vi "_lcod_CFX.vi"(4 "RequestTargetAddress":string="rabbit@SMT-001", 6 "RequestNetworkUri":string="amqp://localhost:5672/#/connections.com", 7 "cmd":T2, 8 "Error In":errorcluster caption="错误输入", 9 "in_str":string, 10 "CFXHandle":string="SDC.SMT.001", 11 "CfxData":T1) -> (0 "Error Out":errorcluster caption="错误输出", 2 "MessageName":string, 3 "new reference":refnum<k24>)   [LabVIEW 2025]
uses:
  ctl/CfxTopic-cmd.ctl
  CFX_dll/CFX.dll
  ctl/CFX_data.ctl
  <vilib>/Utility/error.llb/Trim Whitespace One-Sided.vi
panel:
  out "FaultOccurrenceId":string
  out "ToJson":string
  out "Message":string
  in  "Uri":string="amqp://localhost:5672/#/connections.com:5672"
  # "EndpointInformation/RequestResult/SupportedTopics"
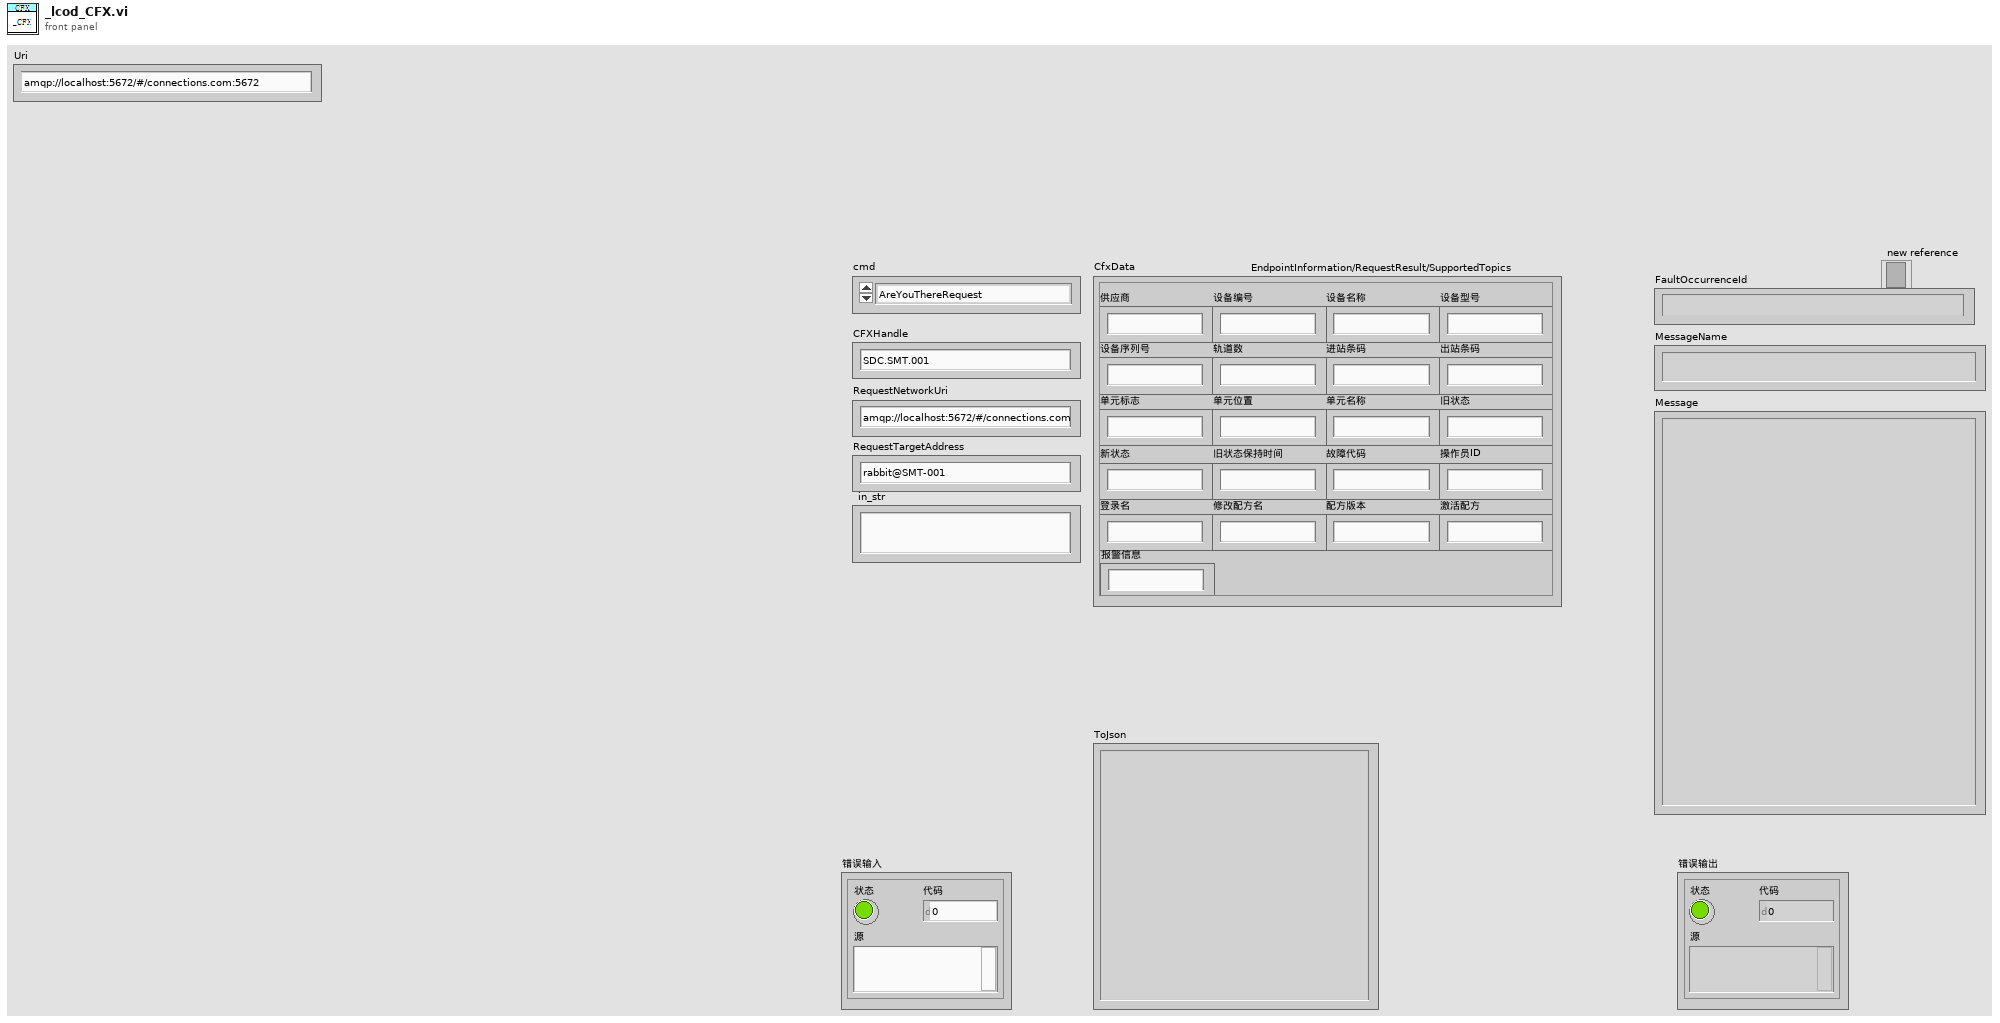
[diagram p1: front panel]
types:
  T1 = typedef "CFX_data.ctl" = cluster{"Vendor":string, "UniqueIdentifier":string, "FriendlyName":string, "ModelNumber":string, "SerialNumber":string, "NumberofLanes":string, "CodeIn":string, "CodeOut":string, "Unitldentifer":string, "PositionNumber":string, "PositionName":string, "OldState":string, "NewState":string, "OldStateDuration":string, "Faultcode":string, "Operatorldentifer":string, "LoginName":string, "RecipeName":string, "Revision":string, "Activate formula":string, "Description":string}
  T2 = typedef "CfxTopic-cmd.ctl" = enum16{"AreYouThereRequest", "AreYouThereResponse", "EndpointConnected", "EndpointShuttingDown", "GetEndpointInformationRequest", "GetEndpointInformationResponse", "Heartbeat", "NotSupportedResponse", "WhoIsThereRequest", "WhoIsThereResponse", "UnitArrived", "UnitsDeparted", "StationStateChanged", "FaultOccurred", "FaultCleared", "OperatorActivated", "OperatorDeactivated", "RecipeModified", "RecipeActived", "ActivateRecipeRequest", "ActivateRecipeResponse"}
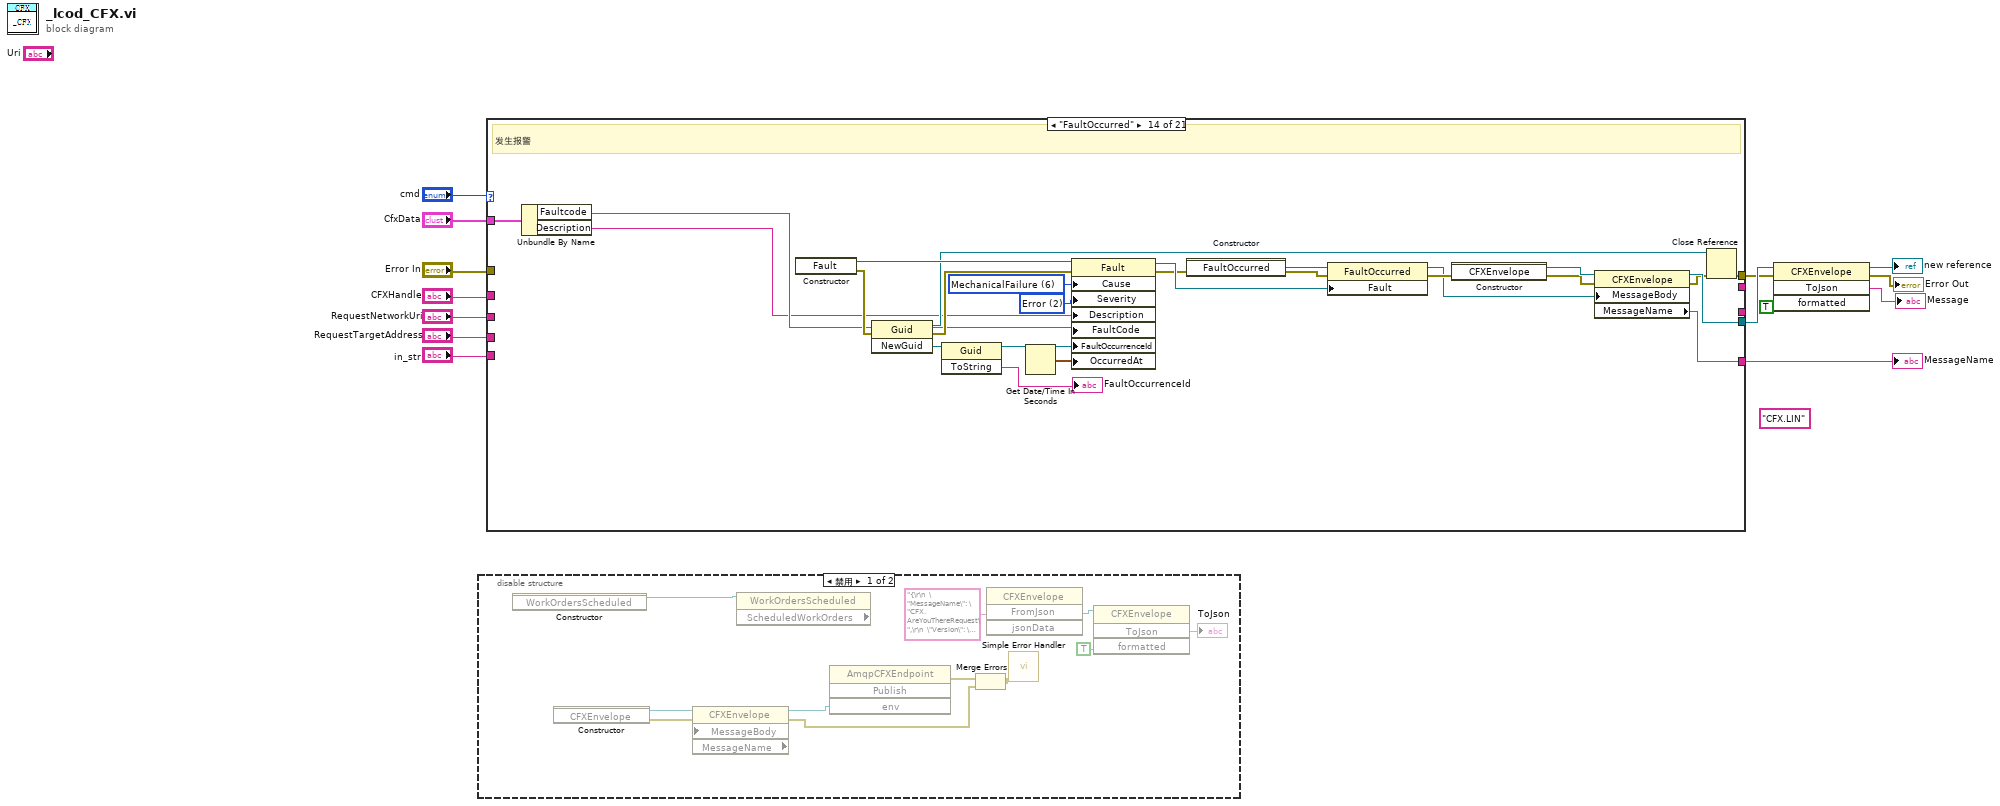
[diagram p0: block diagram]
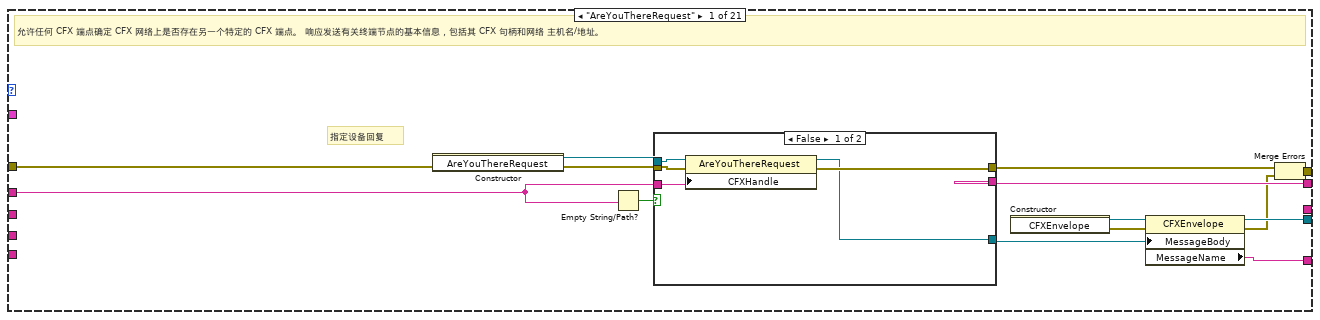
[diagram p3: hidden frame]
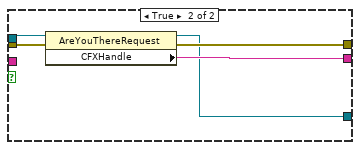
[diagram p4: hidden frame]
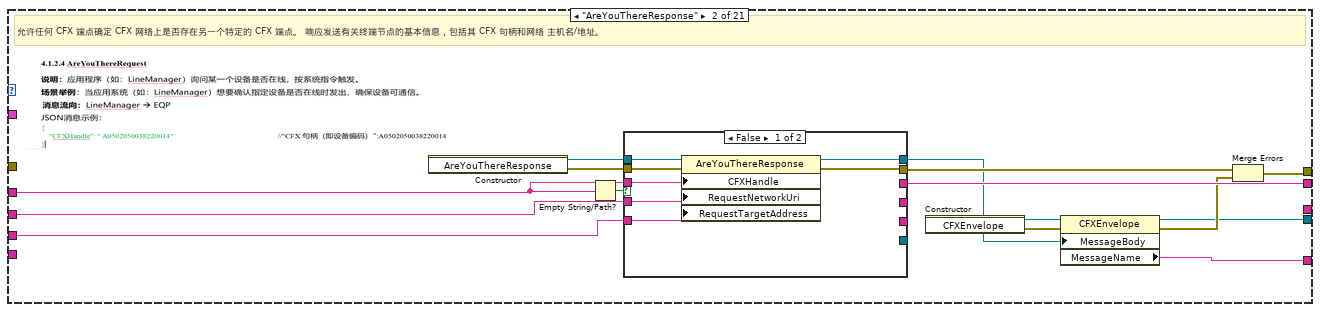
[diagram p5: hidden frame]
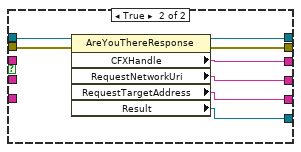
[diagram p6: hidden frame]
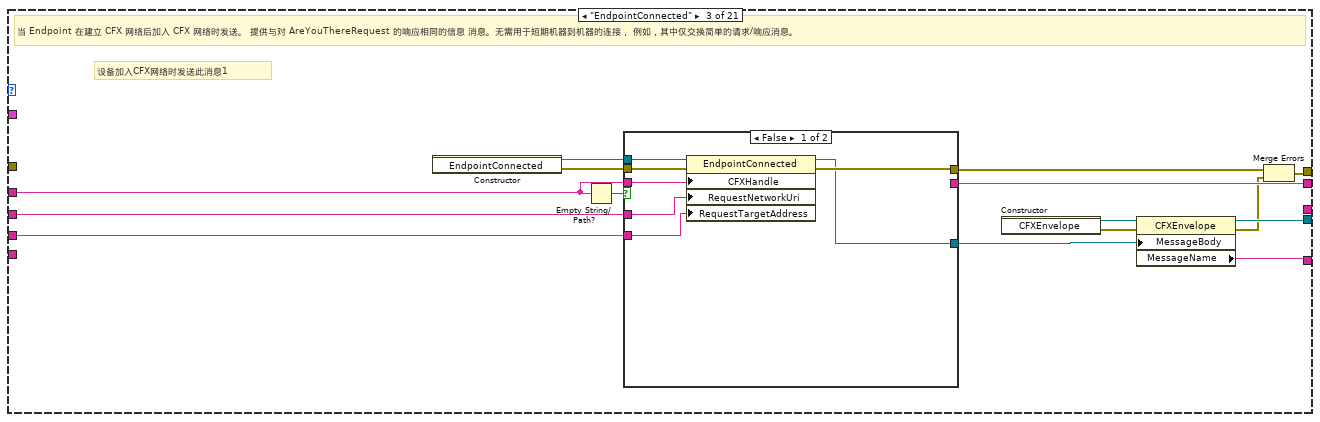
[diagram p7: hidden frame]
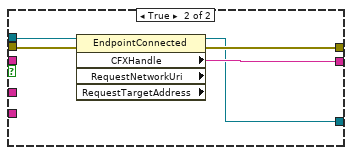
[diagram p8: hidden frame]
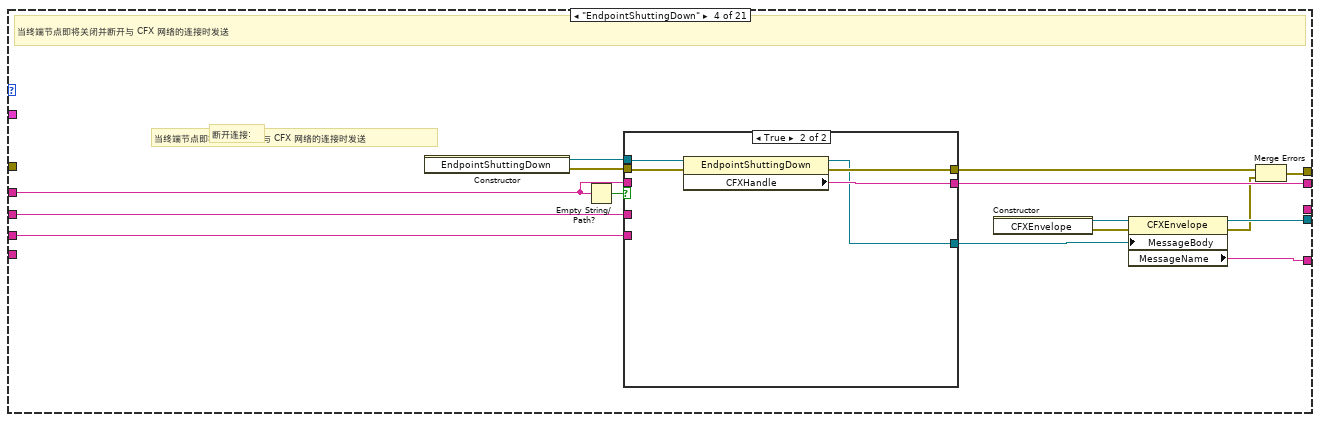
[diagram p9: hidden frame]
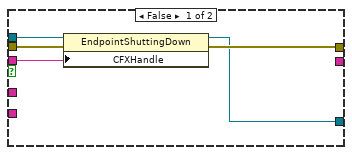
[diagram p10: hidden frame]
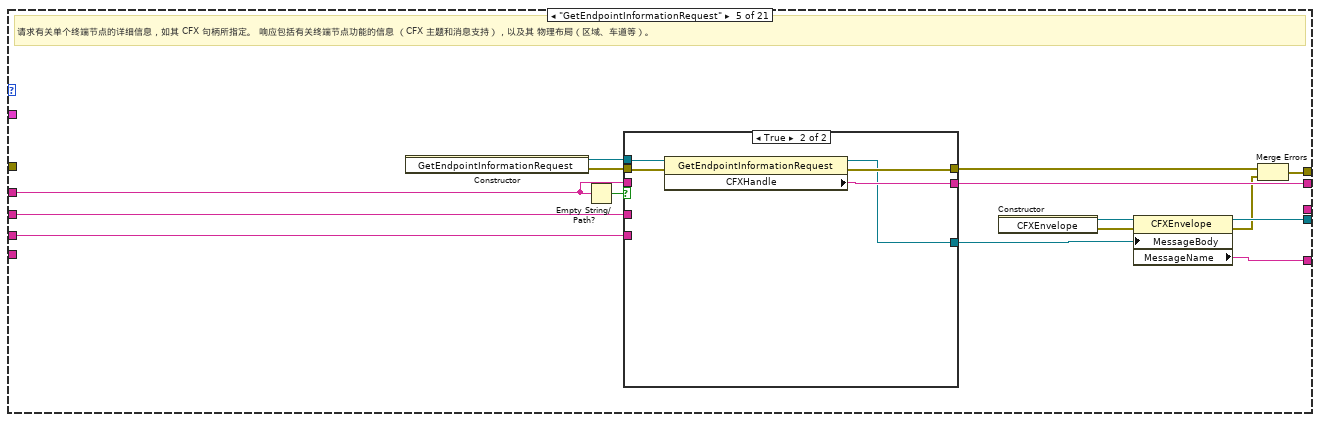
[diagram p11: hidden frame]
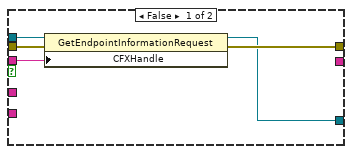
[diagram p12: hidden frame]
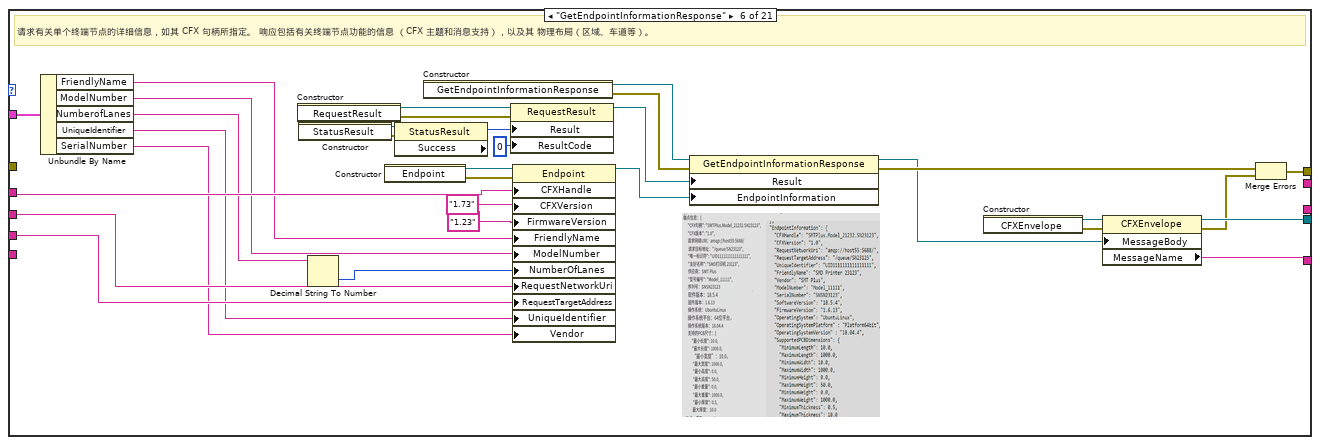
[diagram p13: hidden frame]
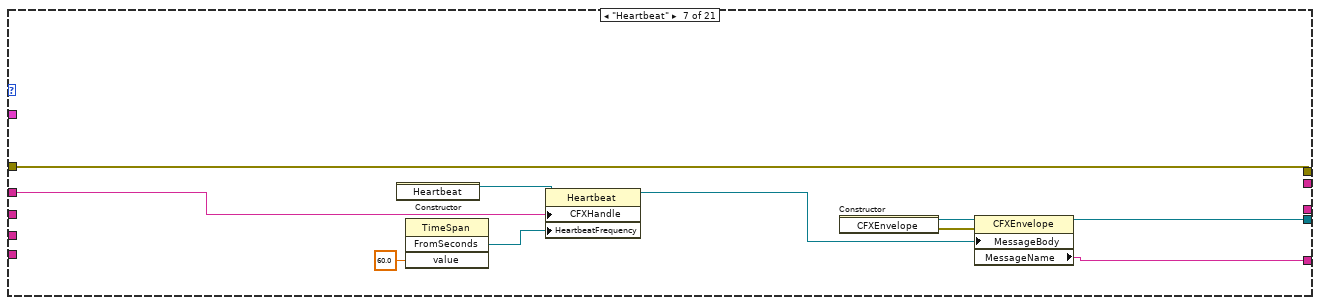
[diagram p14: hidden frame]
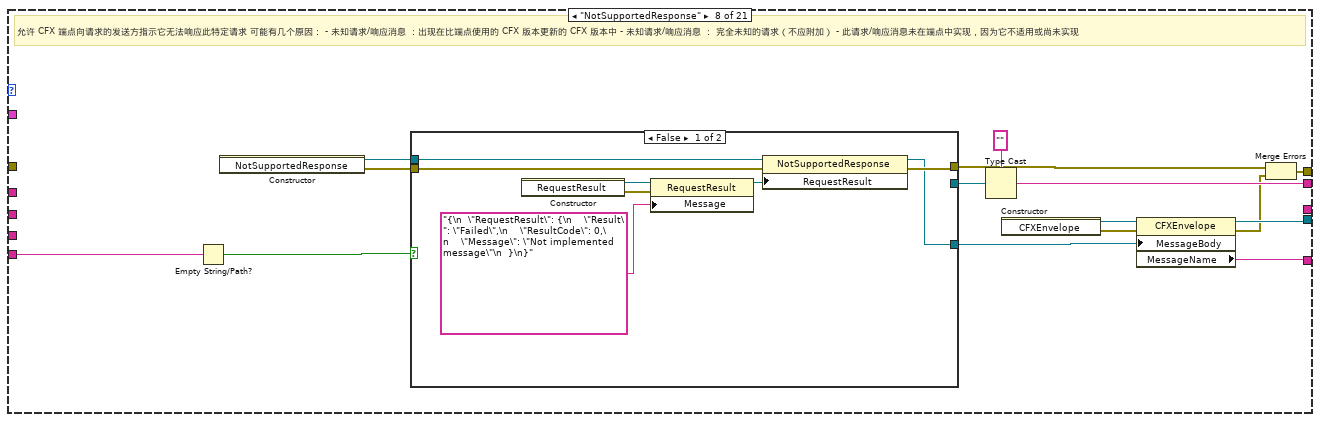
[diagram p15: hidden frame]
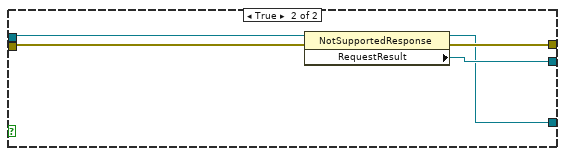
[diagram p16: hidden frame]
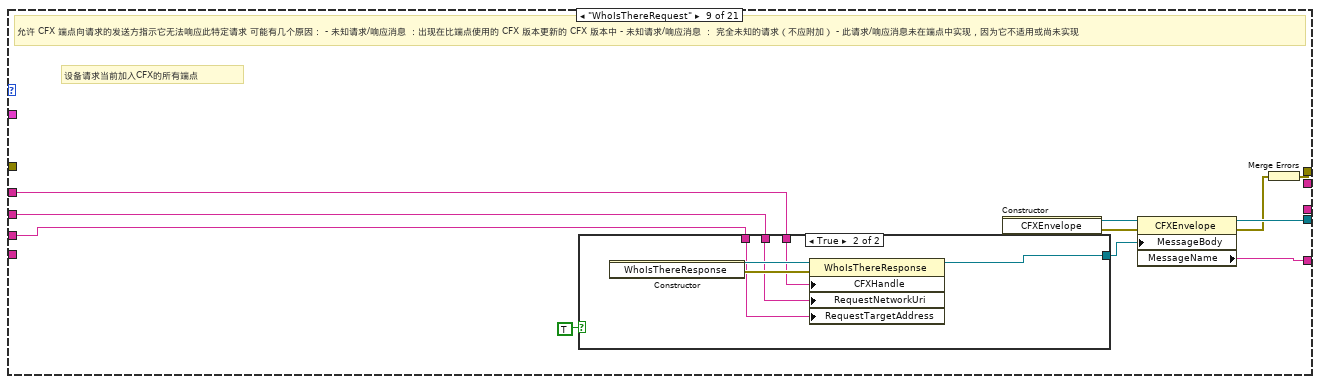
[diagram p17: hidden frame]
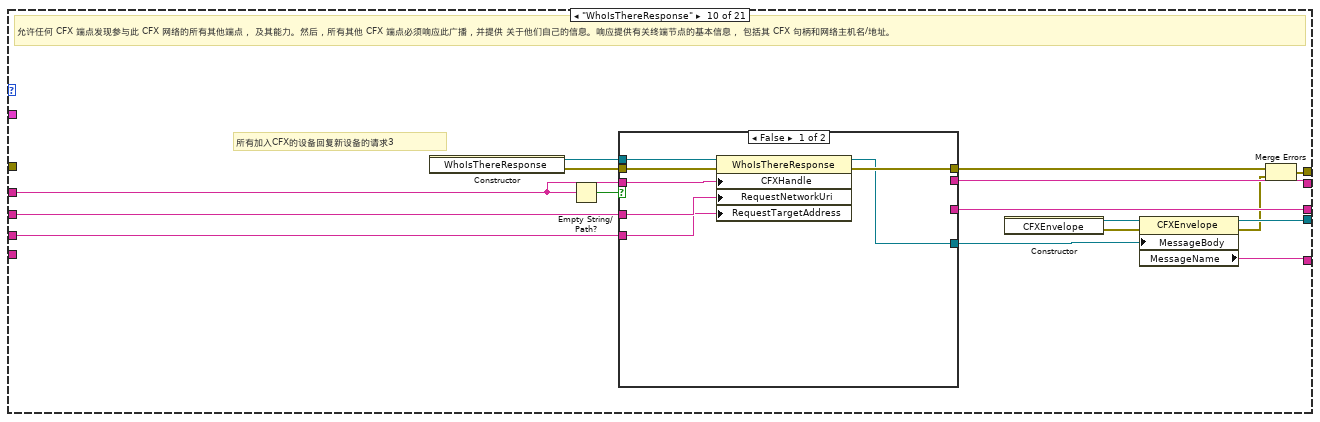
[diagram p19: hidden frame]
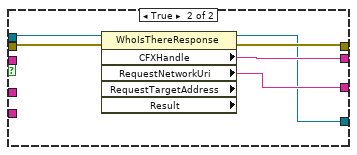
[diagram p20: hidden frame]
diagram:
  (unwired) "CFX.LIN" ("messageType")
  n1 = disable-structure shown="禁用" {
    frame Disabled {
      n2 = constructor class="WorkOrdersScheduled"() -> (reference out=w25:refnum<k24>)  [unwired: 3 in, 2 out]
      n3 = constructor class="CFXEnvelope"() -> (reference out=w22:refnum<k24>, error out=w21:errorcluster)  [unwired: 3 in, 1 out]
      n4 = property class="CFXEnvelope" props=["MessageBody", "MessageName"](reference=w22, error in=w21) -> (reference out=w20:refnum<k24>, error out=w24:errorcluster)  [unwired: 1 in, 1 out]
      n5 = property class="WorkOrdersScheduled" props=["ScheduledWorkOrders"](reference=w25) -> ()  [unwired: 1 in, 3 out]
      n6 = invoke class="AmqpCFXEndpoint" method="Publish"("env"=w20) -> (error out=w19:errorcluster)  [unwired: 3 in, 3 out]
      n7 = Merge Errors(w19, w24) -> (w23:errorcluster)
      n8 = invoke class="CFXEnvelope" method="FromJson"("jsonData"="{\r\n  \"MessageName\": \"CFX.AreYouThereRequest\",\r\n  \"Version\": \"1.75\",\r\n  \"TimeStamp\": \"2025-10-18T15:23:20.890711+08:00\",\r\n  \"UniqueID\": \"92a07db6-b3a6-406f-a014-7739e04793a1\",\r\n  \"Source\": null,\r\n  \"Target\": null,\r\n  \"RequestID\": null,\r\n  \"MessageBody\": {\n\n  \"$type\": \"CFX.AreYouThereRequest, CFX\",\r\n    \"CFXHandle\": \"SDC.SMT.001\"\n\r\n  }\r\n}" ("ToJson")) -> ("FromJson"=w18:refnum<k24>)  [unwired: 3 in, 3 out]
      n9 = call <vilib>:"Simple Error Handler.vi"("error in (no error)"=w23) -> ()  [unwired: 4 in, 5 out]
      n10 = invoke class="CFXEnvelope" method="ToJson"(reference=w18, "formatted"=TRUE) -> ("ToJson"=→"ToJson":string)  [unwired: 2 in, 3 out]
    }
    frame Enabled {
    }
  }
  n11 = case shown="\"FaultOccurred\"" "cmd" {
    tunnel: [w36 w61 w92 w119 w144 _ _ w208 _ w252 _ _ _ _ _ _ _ _ _ _ _] -> _
    tunnel: "CFXHandle" -> [w35 w60 w90 w117 w142 w165 w196 _ w228 w255 _ _ _ _ _ _ _ _ _ _ _]
    tunnel: [w27 w53 w82 w109 w134 w181 w198 w201 w234 w246 w292 w312 w346 w373 w397 w425 w439 w458 w471 w486 w494] -> w4
    tunnel: "Error In" -> [w33 _ _ _ _ _ w198 _ _ _ _ _ _ _ _ _ _ _ w475 _ _]
    tunnel: "RequestTargetAddress" -> [_ w59 w88 w115 w140 w168 _ _ w227 w253 _ _ _ _ _ _ _ _ _ _ _]
    tunnel: "RequestNetworkUri" -> [_ w58 w89 w116 w141 w169 _ _ w229 w254 _ _ _ _ _ _ _ _ _ _ _]
    tunnel: "in_str" -> [_ _ _ _ _ _ _ w209 _ _ _ _ _ _ _ _ _ _ _ _ _]
    tunnel: [_ _ _ _ _ _ _ _ _ w251 _ _ _ _ _ _ _ _ _ _ _] -> _
    tunnel: [w29 w51 w83 w111 w136 w183 w193 w203 w235 w248 w294 w311 w347 w381 w409 w421 w438 w457 w473 w485 w498] -> w6
    tunnel: [w28 w50 w80 w107 w132 w179 w189 w199 w232 w244 w290 w310 w343 w379 w406 w423 w437 w456 w472 w484 w497] -> w8
    tunnel: "CfxData" -> [_ _ _ _ _ w164 _ _ _ _ w280 w308 w342 w378 w405 w420 w436 w453 w470 w483 _]
    frame "AreYouThereRequest" {
      # "指定设备回复"
      # "允许任何 CFX 端点确定 CFX 网络上是否存在另一个特定的 CFX 端点。 响应发送有关终端节点的基本信息，包括其 CFX 句柄和网络 主机名/地址。"
      n12 = constructor class="AreYouThereRequest"(error in=w33) -> (reference out=w38:refnum<k24>, error out=w39:errorcluster)  [unwired: 2 in, 1 out]
      n13 = Empty String/Path?(string/path=w35) -> (empty?=w37:bool)
      n14 = case shown="False" w37 {
        tunnel: w39 -> [w44 w47]
        tunnel: w35 -> [w43 _]
        tunnel: w38 -> [w42 w49]
        tunnel: [_ w48] -> w36
        tunnel: [w41 w46] -> w34
        tunnel: [w40 w45] -> w30
        frame False {
          n15 = property class="AreYouThereRequest"(reference=w42, error in=w44, "CFXHandle"=w43) -> (reference out=w40:refnum<k24>, error out=w41:errorcluster)
        }
        frame True {
          n16 = property class="AreYouThereRequest"(reference=w49, error in=w47) -> (reference out=w45:refnum<k24>, error out=w46:errorcluster, "CFXHandle"=w48:string)
        }
      }
      n17 = constructor class="CFXEnvelope"() -> (reference out=w32:refnum<k24>, error out=w31:errorcluster)  [unwired: 3 in, 1 out]
      n18 = property class="CFXEnvelope"(reference=w32, error in=w31, "MessageBody"=w30) -> (reference out=w29:refnum<k24>, error out=w26:errorcluster, "MessageName"=w28:string)
      n19 = Merge Errors(w34, w26) -> (w27:errorcluster)
    }
    frame "AreYouThereResponse" {
      # "允许任何 CFX 端点确定 CFX 网络上是否存在另一个特定的 CFX 端点。 响应发送有关终端节点的基本信息，包括其 CFX 句柄和网络 主机名/地址。"
      n20 = constructor class="AreYouThereResponse"() -> (reference out=w63:refnum<k24>, error out=w64:errorcluster)  [unwired: 3 in, 1 out]
      n21 = Empty String/Path?(string/path=w60) -> (empty?=w62:bool)
      n22 = case shown="False" w62 {
        tunnel: w64 -> [w71 w77]
        tunnel: w60 -> [w70 _]
        tunnel: w63 -> [w69 w79]
        tunnel: [_ w78] -> w61
        tunnel: w58 -> [w68 _]
        tunnel: w59 -> [w67 _]
        tunnel: [_ w76] -> _
        tunnel: [_ w75] -> _
        tunnel: [_ w74] -> _
        tunnel: [w66 w73] -> w57
        tunnel: [w65 w72] -> w54
        frame False {
          n23 = property class="AreYouThereResponse"(reference=w69, error in=w71, "CFXHandle"=w70, "RequestNetworkUri"=w68, "RequestTargetAddress"=w67) -> (reference out=w65:refnum<k24>, error out=w66:errorcluster)
        }
        frame True {
          n24 = property class="AreYouThereResponse"(reference=w79, error in=w77) -> (reference out=w72:refnum<k24>, error out=w73:errorcluster, "CFXHandle"=w78:string, "RequestNetworkUri"=w76:string, "RequestTargetAddress"=w75:string, "Result"=w74:refnum<k24>)
        }
      }
      n25 = constructor class="CFXEnvelope"() -> (reference out=w56:refnum<k24>, error out=w55:errorcluster)  [unwired: 3 in, 1 out]
      n26 = property class="CFXEnvelope"(reference=w56, error in=w55, "MessageBody"=w54) -> (reference out=w51:refnum<k24>, error out=w52:errorcluster, "MessageName"=w50:string)
      n27 = Merge Errors(w57, w52) -> (w53:errorcluster)
    }
    frame "EndpointConnected" {
      # "设备加入CFX网络时发送此消息1"
      # "当 Endpoint 在建立 CFX 网络后加入 CFX 网络时发送。 提供与对 AreYouThereRequest 的响应相同的信息 消息。无需用于短期机器到机器的连接， 例如，其中仅交换简单的请求/响应消息。"
      n28 = constructor class="EndpointConnected"() -> (reference out=w93:refnum<k24>, error out=w94:errorcluster)  [unwired: 3 in, 1 out]
      n29 = Empty String/Path?(string/path=w90) -> (empty?=w91:bool)
      n30 = case shown="False" w91 {
        tunnel: w94 -> [w101 w105]
        tunnel: w93 -> [w100 w106]
        tunnel: [_ w104] -> w92
        tunnel: w90 -> [w99 _]
        tunnel: w89 -> [w96 _]
        tunnel: w88 -> [w95 _]
        tunnel: [w98 w103] -> w87
        tunnel: [w97 w102] -> w84
        frame False {
          n31 = property class="EndpointConnected"(reference=w100, error in=w101, "CFXHandle"=w99, "RequestNetworkUri"=w96, "RequestTargetAddress"=w95) -> (reference out=w97:refnum<k24>, error out=w98:errorcluster)
        }
        frame True {
          n32 = property class="EndpointConnected" props=["CFXHandle", "RequestNetworkUri", "RequestTargetAddress"](reference=w106, error in=w105) -> (reference out=w102:refnum<k24>, error out=w103:errorcluster, "CFXHandle"=w104:string)  [unwired: 2 out]
        }
      }
      n33 = constructor class="CFXEnvelope"() -> (reference out=w86:refnum<k24>, error out=w85:errorcluster)  [unwired: 3 in, 1 out]
      n34 = property class="CFXEnvelope"(reference=w86, error in=w85, "MessageBody"=w84) -> (reference out=w83:refnum<k24>, error out=w81:errorcluster, "MessageName"=w80:string)
      n35 = Merge Errors(w87, w81) -> (w82:errorcluster)
    }
    frame "EndpointShuttingDown" {
      # "当终端节点即将关闭并断开与 CFX 网络的连接时发送"
      # "断开连接:"
      # "当终端节点即将关闭并断开与 CFX 网络的连接时发送"
      n36 = constructor class="EndpointShuttingDown"() -> (reference out=w120:refnum<k24>, error out=w121:errorcluster)  [unwired: 3 in, 1 out]
      n37 = Empty String/Path?(string/path=w117) -> (empty?=w118:bool)
      n38 = case shown="True" w118 {
        tunnel: w121 -> [w126 w130]
        tunnel: w120 -> [w125 w131]
        tunnel: [_ w129] -> w119
        tunnel: w117 -> [w124 _]
        tunnel: w116 -> [_ _]
        tunnel: w115 -> [_ _]
        tunnel: [w123 w128] -> w114
        tunnel: [w122 w127] -> w110
        frame False {
          n39 = property class="EndpointShuttingDown"(reference=w125, error in=w126, "CFXHandle"=w124) -> (reference out=w122:refnum<k24>, error out=w123:errorcluster)
        }
        frame True {
          n40 = property class="EndpointShuttingDown"(reference=w131, error in=w130) -> (reference out=w127:refnum<k24>, error out=w128:errorcluster, "CFXHandle"=w129:string)
        }
      }
      n41 = constructor class="CFXEnvelope"() -> (reference out=w113:refnum<k24>, error out=w112:errorcluster)  [unwired: 3 in, 1 out]
      n42 = property class="CFXEnvelope"(reference=w113, error in=w112, "MessageBody"=w110) -> (reference out=w111:refnum<k24>, error out=w108:errorcluster, "MessageName"=w107:string)
      n43 = Merge Errors(w114, w108) -> (w109:errorcluster)
    }
    frame "GetEndpointInformationRequest" {
      # "请求有关单个终端节点的详细信息，如其 CFX 句柄所指定。 响应包括有关终端节点功能的信息 （CFX 主题和消息支持），以及其 物理布局（区域、车道等）。"
      n44 = constructor class="GetEndpointInformationRequest"() -> (reference out=w145:refnum<k24>, error out=w146:errorcluster)  [unwired: 3 in, 1 out]
      n45 = Empty String/Path?(string/path=w142) -> (empty?=w143:bool)
      n46 = case shown="True" w143 {
        tunnel: w146 -> [w151 w155]
        tunnel: w145 -> [w150 w156]
        tunnel: [_ w154] -> w144
        tunnel: w142 -> [w149 _]
        tunnel: w141 -> [_ _]
        tunnel: w140 -> [_ _]
        tunnel: [w148 w153] -> w139
        tunnel: [w147 w152] -> w135
        frame False {
          n47 = property class="GetEndpointInformationRequest"(reference=w150, error in=w151, "CFXHandle"=w149) -> (reference out=w147:refnum<k24>, error out=w148:errorcluster)
        }
        frame True {
          n48 = property class="GetEndpointInformationRequest"(reference=w156, error in=w155) -> (reference out=w152:refnum<k24>, error out=w153:errorcluster, "CFXHandle"=w154:string)
        }
      }
      n49 = constructor class="CFXEnvelope"() -> (reference out=w138:refnum<k24>, error out=w137:errorcluster)  [unwired: 3 in, 1 out]
      n50 = property class="CFXEnvelope"(reference=w138, error in=w137, "MessageBody"=w135) -> (reference out=w136:refnum<k24>, error out=w133:errorcluster, "MessageName"=w132:string)
      n51 = Merge Errors(w139, w133) -> (w134:errorcluster)
    }
    frame "GetEndpointInformationResponse" {
      # "请求有关单个终端节点的详细信息，如其 CFX 句柄所指定。 响应包括有关终端节点功能的信息 （CFX 主题和消息支持），以及其 物理布局（区域、车道等）。"
      n52 = Unbundle By Name(w164) -> ("FriendlyName"=w162:string, "ModelNumber"=w161:string, "NumberofLanes"=w160:string, "UniqueIdentifier"=w159:string, "SerialNumber"=w158:string)
      n53 = constructor class="RequestResult"() -> (reference out=w178:refnum<k24>, error out=w177:errorcluster)  [unwired: 3 in, 1 out]
      n54 = constructor class="StatusResult"() -> (reference out=w176:refnum<k24>, error out=w175:errorcluster)  [unwired: 3 in, 1 out]
      n55 = Decimal String To Number(string=w160) -> (number=w157:i32)  [unwired: 2 in, 1 out]
      n56 = constructor class="Endpoint"() -> (reference out=w163:refnum<k24>, error out=w172:errorcluster)  [unwired: 3 in, 1 out]
      n57 = property class="StatusResult"(reference=w176, error in=w175) -> ("Success"=w174:i32)  [unwired: 2 out]
      n58 = constructor class="GetEndpointInformationResponse"() -> (reference out=w187:refnum<k24>, error out=w188:errorcluster)  [unwired: 3 in, 1 out]
      n59 = property on="属性节点" class="RequestResult"(reference=w178, error in=w177, "Result"=w174, "ResultCode"=0) -> (reference out=w167:refnum<k24>)  [unwired: 1 out]
      n60 = property class="Endpoint"(reference=w163, error in=w172, "CFXHandle"=w165, "CFXVersion"="1.73", "FirmwareVersion"="1.23", "FriendlyName"=w162, "ModelNumber"=w161, "NumberOfLanes"=w157, "RequestNetworkUri"=w169, "RequestTargetAddress"=w168, "UniqueIdentifier"=w159, "Vendor"=w158) -> (reference out=w166:refnum<k24>)  [unwired: 1 out]
      n61 = property class="GetEndpointInformationResponse"(reference=w187, error in=w188, "Result"=w167, "EndpointInformation"=w166) -> (reference out=w182:refnum<k24>, error out=w186:errorcluster)
      n62 = constructor class="CFXEnvelope"() -> (reference out=w185:refnum<k24>, error out=w184:errorcluster)  [unwired: 3 in, 1 out]
      n63 = property class="CFXEnvelope"(reference=w185, error in=w184, "MessageBody"=w182) -> (reference out=w183:refnum<k24>, error out=w180:errorcluster, "MessageName"=w179:string)
      n64 = Merge Errors(w186, w180) -> (w181:errorcluster)
    }
    frame "Heartbeat" {
      n65 = constructor class="Heartbeat"() -> (reference out=w197:refnum<k24>)  [unwired: 3 in, 2 out]
      n66 = invoke on="调用节点" class="TimeSpan" method="FromSeconds"("value"=60.0) -> ("FromSeconds"=w191:refnum<k24>)  [unwired: 3 in, 3 out]
      n67 = property class="Heartbeat"(reference=w197, "CFXHandle"=w196, "HeartbeatFrequency"=w191) -> (reference out=w192:refnum<k24>)  [unwired: 1 in, 1 out]
      n68 = constructor class="CFXEnvelope"() -> (reference out=w195:refnum<k24>, error out=w194:errorcluster)  [unwired: 3 in, 1 out]
      n69 = property class="CFXEnvelope"(reference=w195, error in=w194, "MessageBody"=w192) -> (reference out=w193:refnum<k24>, "MessageName"=w189:string)  [unwired: 1 out]
    }
    frame "NotSupportedResponse" {
      # "允许 CFX 端点向请求的发送方指示它无法响应此特定请求 可能有几个原因： - 未知请求/响应消息 ：出现在比端点使用的 CFX 版本更新的 CFX 版本中 - 未知请求/响应消息 ： 完全未知的请求（不应附加） - 此请求/响应消息未在端点中实现，因为它不适用或尚未实现"
      n70 = Empty String/Path?(string/path=w209) -> (empty?=w210:bool)
      n71 = constructor class="NotSupportedResponse"() -> (reference out=w212:refnum<k24>, error out=w213:errorcluster)  [unwired: 3 in, 1 out]
      n72 = case shown="False" w210 {
        tunnel: w213 -> [w221 w225]
        tunnel: w212 -> [w220 w226]
        tunnel: [_ w224] -> w211
        tunnel: [w219 w223] -> w206
        tunnel: [w218 w222] -> w202
        frame False {
          n73 = constructor class="RequestResult"() -> (reference out=w215:refnum<k24>, error out=w214:errorcluster)  [unwired: 3 in, 1 out]
          n74 = property class="RequestResult"(reference=w215, error in=w214, "Message"="{\n  \"RequestResult\": {\n    \"Result\": \"Failed\",\n    \"ResultCode\": 0,\n    \"Message\": \"Not implemented message\"\n  }\n}") -> (reference out=w217:refnum<k24>)  [unwired: 1 out]
          n75 = property class="NotSupportedResponse"(reference=w220, error in=w221, "RequestResult"=w217) -> (reference out=w218:refnum<k24>, error out=w219:errorcluster)
        }
        frame True {
          n76 = property class="NotSupportedResponse"(reference=w226, error in=w225) -> (reference out=w222:refnum<k24>, error out=w223:errorcluster, "RequestResult"=w224:refnum<k24>)
        }
      }
      n77 = Type Cast(type="", x=w211) -> (*(type *) &x=w208:string)
      n78 = constructor class="CFXEnvelope"() -> (reference out=w205:refnum<k24>, error out=w204:errorcluster)  [unwired: 3 in, 1 out]
      n79 = property class="CFXEnvelope"(reference=w205, error in=w204, "MessageBody"=w202) -> (reference out=w203:refnum<k24>, error out=w200:errorcluster, "MessageName"=w199:string)
      n80 = Merge Errors(w206, w200) -> (w201:errorcluster)
    }
    frame "WhoIsThereRequest" {
      # "设备请求当前加入CFX的所有端点"
      # "允许 CFX 端点向请求的发送方指示它无法响应此特定请求 可能有几个原因： - 未知请求/响应消息 ：出现在比端点使用的 CFX 版本更新的 CFX 版本中 - 未知请求/响应消息 ： 完全未知的请求（不应附加） - 此请求/响应消息未在端点中实现，因为它不适用或尚未实现"
      n81 = case shown="True" TRUE {
        tunnel: [_ w238] -> w230
        tunnel: w229 -> [_ w241]
        tunnel: w228 -> [_ w240]
        tunnel: w227 -> [_ w239]
        frame False {
        }
        frame True {
          n82 = constructor class="WhoIsThereResponse"() -> (reference out=w243:refnum<k24>, error out=w242:errorcluster)  [unwired: 3 in, 1 out]
          n83 = property class="WhoIsThereResponse"(reference=w243, error in=w242, "CFXHandle"=w240, "RequestNetworkUri"=w241, "RequestTargetAddress"=w239) -> (reference out=w238:refnum<k24>)  [unwired: 1 out]
        }
      }
      n84 = constructor class="CFXEnvelope"() -> (reference out=w237:refnum<k24>, error out=w236:errorcluster)  [unwired: 3 in, 1 out]
      n85 = property class="CFXEnvelope"(reference=w237, error in=w236, "MessageBody"=w230) -> (reference out=w235:refnum<k24>, error out=w233:errorcluster, "MessageName"=w232:string)
      n86 = Merge Errors(w233) -> (w234:errorcluster)
    }
    frame "WhoIsThereResponse" {
      # "所有加入CFX的设备回复新设备的请求3"
      # "允许任何 CFX 端点发现参与此 CFX 网络的所有其他端点， 及其能力。然后，所有其他 CFX 端点必须响应此广播，并提供 关于他们自己的信息。响应提供有关终端节点的基本信息， 包括其 CFX 句柄和网络主机名/地址。"
      n87 = constructor class="WhoIsThereResponse"() -> (reference out=w258:refnum<k24>, error out=w259:errorcluster)  [unwired: 3 in, 1 out]
      n88 = Empty String/Path?(string/path=w255) -> (empty?=w257:bool)
      n89 = case shown="False" w257 {
        tunnel: w259 -> [w266 w271]
        tunnel: w258 -> [w265 w272]
        tunnel: [w264 w270] -> w256
        tunnel: w255 -> [w263 _]
        tunnel: w254 -> [w262 _]
        tunnel: w253 -> [w261 _]
        tunnel: [_ w269] -> w252
        tunnel: [_ w268] -> w251
        tunnel: [w260 w267] -> w247
        frame False {
          n90 = property class="WhoIsThereResponse"(reference=w265, error in=w266, "CFXHandle"=w263, "RequestNetworkUri"=w262, "RequestTargetAddress"=w261) -> (reference out=w260:refnum<k24>, error out=w264:errorcluster)
        }
        frame True {
          n91 = property class="WhoIsThereResponse" props=["CFXHandle", "RequestNetworkUri", "RequestTargetAddress", "Result"](reference=w272, error in=w271) -> (reference out=w267:refnum<k24>, error out=w270:errorcluster, "CFXHandle"=w269:string, "RequestNetworkUri"=w268:string)  [unwired: 2 out]
        }
      }
      n92 = constructor class="CFXEnvelope"() -> (reference out=w250:refnum<k24>, error out=w249:errorcluster)  [unwired: 3 in, 1 out]
      n93 = property class="CFXEnvelope"(reference=w250, error in=w249, "MessageBody"=w247) -> (reference out=w248:refnum<k24>, error out=w245:errorcluster, "MessageName"=w244:string)
      n94 = Merge Errors(w256, w245) -> (w246:errorcluster)
    }
    frame "UnitArrived" {
      (unwired) "17163000009047XD06A25041900001" ("UnitIdentifier")
      (unwired) 1 ("PositionNumber")
      # "{\n  \"UnitCount\": 2, \t\t\t\t\t\t\t\t\t// 单元数量：2\n  \"Units\": [\n    {\n      \"UnitIdentifier\": \"17163000009047XD06A25041900001\",\t \t// 位置号1的小板条码：17163000009047XD06A25041900001（最小生产单元条码信息）\n      \"PositionNumber\": 1, \t\t\t\t\t\t\t// 位置编号：1（位置编号参考位置号编码规则上报，按流板方向“从左到右，从上到下”）\n      \"PositionName\": \"PostAOI\", \t\t\t\t\t\t// 站点名称PostAOI（注意：此处上报的是当前站点名称，如炉后AOI，上报PostAOI）\n     \n    },\n    {\n      \"UnitIdentifier\": \"17163000009047XD06A25041900002\", \t\t// 位置号2的小板条码：17163000009047XD06A25041900001（最小生产单元条码信息）\n      \"PositionNumber\": 2, \t\t\t\t\t\t\t// 位置编号：2\n     \"PositionName\": \"PostAOI\", \t\t\t\t\t\t// 站点名称：PostAOI    \n    }\n  ]\n}"
      # "单元到达。当一组生产单元到达设备时发送此消息（到达感应器触发时）。"
      n95 = Unbundle By Name(w280) -> ("CodeIn"=w274:string, "PositionNumber"=w279:string, "PositionName"=w277:string)
      n96 = call <vilib>:"Trim Whitespace.vi"("string"=w274) -> ("trimmed string"=w273:string)  [unwired: 1 in]
      n97 = Empty String/Path?(string/path=w273) -> (empty?=w275:bool)
      n98 = case shown="True" w275 {
        tunnel: [w298 w299] -> w276
        tunnel: w273 -> [w298 _]
        frame False {
        }
        frame True {
          n99 = call "lcod Virtual barcode.vi"("cmd"=enum16{"init", "set", "get"}."set") -> ("code"=w299:string)  [unwired: 9 in, 1 out]
        }
      }
      n100 = Decimal String To Number(string=w279) -> (number=w278:i32)  [unwired: 2 in, 1 out]
      n101 = constructor class="UnitPosition"() -> (reference out=w289:refnum<k24>, error out=w281:errorcluster)  [unwired: 3 in, 1 out]
      n102 = constructor class="UnitsArrived"() -> (reference out=w288:refnum<k24>)  [unwired: 3 in, 2 out]
      n103 = property on="属性节点" class="UnitsArrived"(reference=w288) -> (reference out=w285:refnum<k24>, error out=w283:errorcluster, "Units"=w284:refnum<k24>)  [unwired: 1 in]
      n104 = property class="UnitPosition"(reference=w289, error in=w281, "UnitIdentifier"=w276, "PositionNumber"=w278, "PositionName"=w277) -> (reference out=w286:refnum<k24>)  [unwired: 1 out]
      n105 = invoke class="List`1[[CFX.Structures.UnitPosi" method="Add"(reference=w284, error in=w283, "item"=w286) -> (reference out=w287:refnum<k24>, error out=w282:errorcluster)  [unwired: 1 in, 2 out]
      n106 = property class="UnitsArrived"(reference=w285, error in=w282, "Units"=w287) -> (reference out=w293:refnum<k24>, error out=w297:errorcluster)
      n107 = constructor class="CFXEnvelope"() -> (reference out=w296:refnum<k24>, error out=w295:errorcluster)  [unwired: 3 in, 1 out]
      n108 = property class="CFXEnvelope"(reference=w296, error in=w295, "MessageBody"=w293) -> (reference out=w294:refnum<k24>, error out=w291:errorcluster, "MessageName"=w290:string)
      n109 = Merge Errors(w297, w291) -> (w292:errorcluster)
    }
    frame "UnitsDeparted" {
      w301 = 0 items=["Pass", "Fail", "Scrap", "Skip"] ("Status")
      (unwired) "17163000009047XD06A25041900001" ("UnitIdentifier")
      (unwired) 1 ("PositionNumber")
      n110 = Unbundle By Name(w308) -> ("CodeOut"=w302:string, "PositionNumber"=w307:string, "PositionName"=w305:string)
      n111 = Empty String/Path?(string/path=w302) -> (empty?=w304:bool)
      n112 = case shown="True" w304 {
        tunnel: [w327 w329] -> w303
        tunnel: w302 -> [w327 _]
        frame False {
        }
        frame True {
          n113 = call "lcod Virtual barcode.vi"("cmd"=enum16{"init", "set", "get"}."get") -> ("Virtual_barcode[]"=w329:string)  [unwired: 9 in, 1 out]
        }
      }
      n114 = Decimal String To Number(string=w307) -> (number=w306:i32)  [unwired: 2 in, 1 out]
      n115 = constructor class="UnitsDeparted"() -> (reference out=w320:refnum<k24>, error out=w309:errorcluster)  [unwired: 3 in, 1 out]
      n116 = constructor class="UnitPosition"() -> (reference out=w321:refnum<k24>, error out=w313:errorcluster)  [unwired: 3 in, 1 out]
      n117 = property on="属性节点" class="UnitsDeparted"(reference=w320, error in=w309) -> (reference out=w317:refnum<k24>, error out=w315:errorcluster, "Units"=w316:refnum<k24>)
      n118 = property class="UnitPosition"(reference=w321, error in=w313, "UnitIdentifier"=w303, "PositionNumber"=w306, "PositionName"=w305, "Status"=w301) -> (reference out=w318:refnum<k24>)  [unwired: 1 out]
      n119 = invoke class="List`1[[CFX.Structures.UnitPosi" method="Add"(reference=w316, error in=w315, "item"=w318) -> (reference out=w319:refnum<k24>, error out=w314:errorcluster)  [unwired: 1 in, 2 out]
      n120 = property class="UnitsDeparted"(reference=w317, error in=w314, "Units"=w319) -> (reference out=w323:refnum<k24>, error out=w326:errorcluster)
      n121 = constructor class="CFXEnvelope"() -> (reference out=w325:refnum<k24>, error out=w324:errorcluster)  [unwired: 3 in, 1 out]
      n122 = property class="CFXEnvelope"(reference=w325, error in=w324, "MessageBody"=w323) -> (reference out=w311:refnum<k24>, error out=w322:errorcluster, "MessageName"=w310:string)
      n123 = Merge Errors(w326, w322) -> (w312:errorcluster)
    }
    frame "StationStateChanged" {
      (unwired) 123.0 ("value")
      # "设备状态"
      n124 = Unbundle By Name(w342) -> ("OldState"=w341:string, "NewState"=w338:string, "Faultcode"=w336:string, "Operatorldentifer"=w335:string)
      n125 = Decimal String To Number(string=w341) -> (number=w340:i32)  [unwired: 2 in, 1 out]
      n126 = Decimal String To Number(string=w338) -> (number=w330:i32)  [unwired: 2 in, 1 out]
      n127 = Decimal String To Number(string=w335) -> (number=w334:i32)  [unwired: 2 in, 1 out]
      n128 = disable-structure shown="已启用" {
        disable-tunnel: w340 -> [w355 w361]
        disable-tunnel: [w354 w361] -> w339
        frame Disabled {
          n129 = case shown="3" w355 {
            tunnel: [0 ("OldState") w357 w358 w359 w360] -> w354
            frame 0, Default {
            }
            frame 1 {
              w357 = 1000 items=["PRD"=1000, "PRD_RegularWork"=1100, "PRD_WorkForThirdParties"=1200, "PRD_Rework"=1300, "PRD_Engineering"=1400, "SBY"=2000, "SBY_NoOperator"=2100, "SBY_NoProduct"=2200, "SBY_NoProductBlocked"=2201, "SBY_NoProductStarved"=2202, "SBY_NoSupportTool"=2300, "SBY_AssociatedClusterModuleDown"=2400, "SBY_NoHost"=2500, "ENG"=3000, "ENG_ProcessExperiments"=3100, "ENG_EquipmentExperiments"=3200, "SDT"=4000, "SDT_UserMaintenanceDelay"=4100, "SDT_SuppliedMaintenanceDelay"=4200, "SDT_PreventiveMaintenance"=4300, "SDT_ChangeOfConsumables"=4400, "SDT_Setup"=4500, "SDT_ProductionTest"=4600, "SDT_FacilitiesRelated"=4700, "USD"=5000, "USD_UserMaintentanceDelay"=5100, "USD_SuppliedMaintenanceDelay"=5200, "USD_Repair"=5300, "USD_OutOfSpecInputMaterial"=5400, "USD_ChangeOfConsumables"=5500, "USD_FacilitiesRelated"=5600, "NST"=6000, "NST_UnworkedShifts"=6100, "NST_EquipmentInstallation"=6200, "NST_EquipmentModifications"=6300, "NST_OfflineTraining"=6400, "NST_ShutdownAndStartup"=6500] ("OldState")
            }
            frame 2 {
              w358 = 2000 items=["PRD"=1000, "PRD_RegularWork"=1100, "PRD_WorkForThirdParties"=1200, "PRD_Rework"=1300, "PRD_Engineering"=1400, "SBY"=2000, "SBY_NoOperator"=2100, "SBY_NoProduct"=2200, "SBY_NoProductBlocked"=2201, "SBY_NoProductStarved"=2202, "SBY_NoSupportTool"=2300, "SBY_AssociatedClusterModuleDown"=2400, "SBY_NoHost"=2500, "ENG"=3000, "ENG_ProcessExperiments"=3100, "ENG_EquipmentExperiments"=3200, "SDT"=4000, "SDT_UserMaintenanceDelay"=4100, "SDT_SuppliedMaintenanceDelay"=4200, "SDT_PreventiveMaintenance"=4300, "SDT_ChangeOfConsumables"=4400, "SDT_Setup"=4500, "SDT_ProductionTest"=4600, "SDT_FacilitiesRelated"=4700, "USD"=5000, "USD_UserMaintentanceDelay"=5100, "USD_SuppliedMaintenanceDelay"=5200, "USD_Repair"=5300, "USD_OutOfSpecInputMaterial"=5400, "USD_ChangeOfConsumables"=5500, "USD_FacilitiesRelated"=5600, "NST"=6000, "NST_UnworkedShifts"=6100, "NST_EquipmentInstallation"=6200, "NST_EquipmentModifications"=6300, "NST_OfflineTraining"=6400, "NST_ShutdownAndStartup"=6500] ("OldState")
            }
            frame 3 {
              w359 = 5000 items=["PRD"=1000, "PRD_RegularWork"=1100, "PRD_WorkForThirdParties"=1200, "PRD_Rework"=1300, "PRD_Engineering"=1400, "SBY"=2000, "SBY_NoOperator"=2100, "SBY_NoProduct"=2200, "SBY_NoProductBlocked"=2201, "SBY_NoProductStarved"=2202, "SBY_NoSupportTool"=2300, "SBY_AssociatedClusterModuleDown"=2400, "SBY_NoHost"=2500, "ENG"=3000, "ENG_ProcessExperiments"=3100, "ENG_EquipmentExperiments"=3200, "SDT"=4000, "SDT_UserMaintenanceDelay"=4100, "SDT_SuppliedMaintenanceDelay"=4200, "SDT_PreventiveMaintenance"=4300, "SDT_ChangeOfConsumables"=4400, "SDT_Setup"=4500, "SDT_ProductionTest"=4600, "SDT_FacilitiesRelated"=4700, "USD"=5000, "USD_UserMaintentanceDelay"=5100, "USD_SuppliedMaintenanceDelay"=5200, "USD_Repair"=5300, "USD_OutOfSpecInputMaterial"=5400, "USD_ChangeOfConsumables"=5500, "USD_FacilitiesRelated"=5600, "NST"=6000, "NST_UnworkedShifts"=6100, "NST_EquipmentInstallation"=6200, "NST_EquipmentModifications"=6300, "NST_OfflineTraining"=6400, "NST_ShutdownAndStartup"=6500] ("OldState")
            }
            frame 4 {
              w360 = 6000 items=["PRD"=1000, "PRD_RegularWork"=1100, "PRD_WorkForThirdParties"=1200, "PRD_Rework"=1300, "PRD_Engineering"=1400, "SBY"=2000, "SBY_NoOperator"=2100, "SBY_NoProduct"=2200, "SBY_NoProductBlocked"=2201, "SBY_NoProductStarved"=2202, "SBY_NoSupportTool"=2300, "SBY_AssociatedClusterModuleDown"=2400, "SBY_NoHost"=2500, "ENG"=3000, "ENG_ProcessExperiments"=3100, "ENG_EquipmentExperiments"=3200, "SDT"=4000, "SDT_UserMaintenanceDelay"=4100, "SDT_SuppliedMaintenanceDelay"=4200, "SDT_PreventiveMaintenance"=4300, "SDT_ChangeOfConsumables"=4400, "SDT_Setup"=4500, "SDT_ProductionTest"=4600, "SDT_FacilitiesRelated"=4700, "USD"=5000, "USD_UserMaintentanceDelay"=5100, "USD_SuppliedMaintenanceDelay"=5200, "USD_Repair"=5300, "USD_OutOfSpecInputMaterial"=5400, "USD_ChangeOfConsumables"=5500, "USD_FacilitiesRelated"=5600, "NST"=6000, "NST_UnworkedShifts"=6100, "NST_EquipmentInstallation"=6200, "NST_EquipmentModifications"=6300, "NST_OfflineTraining"=6400, "NST_ShutdownAndStartup"=6500] ("OldState")
            }
          }
        }
        frame Enabled {
        }
      }
      n130 = Empty String/Path?(string/path=w336) -> (empty?=w337:bool)
      n131 = case shown="False" w337 {
        tunnel: [w365 w368] -> w353
        tunnel: w336 -> [w362 _]
        frame False {
          w364 = 2 items=["Information", "Warning", "Error", "Alarm"] ("Severity")
          w366 = 6 items=["LoadError", "UnloadError", "AutoSafetyStop", "SafetyStop", "QualityCheck", "RemoteStop", "MechanicalFailure", "SoftwareFailure", "PowerFailure", "MissingDocumentation", "Refill", "MsdExpired", "MaterialExpired", "MissingComponent", "ElectricalFailure", "ServicesFailure", "ProcessError", "RejectedComponent"] ("Cause")
          n132 = constructor class="Fault"() -> (reference out=w367:refnum<k24>, error out=w363:errorcluster)  [unwired: 3 in, 1 out]
          n133 = property class="Fault"(reference=w367, error in=w363, "Cause"=w366, "Severity"=w364, "FaultCode"=w362) -> (reference out=w365:refnum<k24>)  [unwired: 1 out]
        }
        frame True {
          n134 = constructor class="Fault"() -> (reference out=w368:refnum<k24>)  [unwired: 3 in, 2 out]
        }
      }
      n135 = To Double Precision Float(number=w334) -> (double precision float=w333:dbl)
      n136 = constructor class="StationStateChanged"() -> (reference out=w348:refnum<k24>, error out=w349:errorcluster)  [unwired: 3 in, 1 out]
      n137 = invoke on="调用节点" class="TimeSpan" method="FromSeconds"("value"=w333) -> (reference out=w331:refnum<k24>, "FromSeconds"=w352:refnum<k24>)  [unwired: 3 in, 2 out]
      n138 = property on="属性节点" class="StationStateChanged"(reference=w348, error in=w349, "OldState"=w339, "OldStateDuration"=w352, "NewState"=w330, "RelatedFault"=w353) -> (reference out=w344:refnum<k24>, error out=w345:errorcluster)
      n139 = Close Reference(reference=w331, error in (no error)=w345) -> (error out=w332:errorcluster)
      n140 = constructor class="CFXEnvelope"(error in=w332) -> (reference out=w351:refnum<k24>, error out=w350:errorcluster)  [unwired: 2 in, 1 out]
      n141 = property on="属性节点" class="CFXEnvelope"(reference=w351, error in=w350, "MessageBody"=w344) -> (reference out=w347:refnum<k24>, error out=w346:errorcluster, "MessageName"=w343:string)
    }
    frame "FaultOccurred" {
      w390 = 2 items=["Information", "Warning", "Error", "Alarm"] ("Severity")
      w391 = 6 items=["LoadError", "UnloadError", "AutoSafetyStop", "SafetyStop", "QualityCheck", "RemoteStop", "MechanicalFailure", "SoftwareFailure", "PowerFailure", "MissingDocumentation", "Refill", "MsdExpired", "MaterialExpired", "MissingComponent", "ElectricalFailure", "ServicesFailure", "ProcessError", "RejectedComponent"] ("Cause")
      # "发生报警"
      n142 = Unbundle By Name(w378) -> ("Faultcode"=w377:string, "Description"=w369:string)
      n143 = constructor class="Fault"() -> (reference out=w384:refnum<k24>, error out=w383:errorcluster)  [unwired: 3 in, 1 out]
      n144 = invoke class="Guid" method="NewGuid"(error in=w383) -> (reference out=w375:refnum<k24>, error out=w382:errorcluster, "NewGuid"=w371:refnum<k24>)  [unwired: 2 in]
      n145 = invoke on="调用节点" class="Guid" method="ToString"(reference=w371) -> (reference out=w370:refnum<k24>, "ToString"=→"FaultOccurrenceId":string)  [unwired: 2 in, 1 out]
      n146 = Get Date/Time In Seconds() -> (seconds since 1Jan1904=w376:timestamp)
      n147 = property class="Fault"(reference=w384, error in=w382, "Cause"=w391, "Severity"=w390, "Description"=w369, "FaultCode"=w377, "FaultOccurrenceId"=w370, "OccurredAt"=w376) -> (reference out=w392:refnum<k24>, error out=w387:errorcluster)
      n148 = constructor class="FaultOccurred"(error in=w387) -> (reference out=w393:refnum<k24>, error out=w386:errorcluster)  [unwired: 2 in, 1 out]
      n149 = property on="属性节点" class="FaultOccurred"(reference=w393, error in=w386, "Fault"=w392) -> (reference out=w380:refnum<k24>, error out=w385:errorcluster)
      n150 = constructor class="CFXEnvelope"(error in=w385) -> (reference out=w389:refnum<k24>, error out=w388:errorcluster)  [unwired: 2 in, 1 out]
      n151 = property on="属性节点" class="CFXEnvelope"(reference=w389, error in=w388, "MessageBody"=w380) -> (reference out=w381:refnum<k24>, error out=w374:errorcluster, "MessageName"=w379:string)
      n152 = Close Reference(reference=w375, error in (no error)=w374) -> (error out=w373:errorcluster)
    }
    frame "FaultCleared" {
      # "清除报警"
      n153 = Unbundle By Name(w405) -> ("Operatorldentifer"=w404:string, "LoginName"=w403:string)
      n154 = constructor class="Operator"() -> (reference out=w415:refnum<k24>, error out=w414:errorcluster)  [unwired: 3 in, 1 out]
      n155 = property class="Operator"(reference=w415, error in=w414, "OperatorIdentifier"=w404, "LoginName"=w403) -> (reference out=w416:refnum<k24>, error out=w408:errorcluster)
      n156 = constructor class="FaultCleared"(error in=w408) -> (reference out=w417:refnum<k24>, error out=w395:errorcluster)  [unwired: 2 in, 1 out]
      n157 = property on="FaultOccurrenceId" class="Str"(error in=w395) -> (error out=w394:errorcluster, "Value"=w402:string)  [unwired: 1 in, 1 out]
      n158 = invoke on="调用节点" class="Guid" method="TryParse"(error in=w394, "input"=w402) -> (reference out=w399:refnum<k24>, error out=w400:errorcluster, "result"=w401:refnum<k24>)  [unwired: 3 in, 2 out]
      n159 = property on="属性节点" class="FaultCleared"(reference=w417, error in=w400, "Operator"=w416, "FaultOccurrenceId"=w401) -> (reference out=w407:refnum<k24>, error out=w411:errorcluster)
      n160 = constructor class="CFXEnvelope"(error in=w411) -> (reference out=w413:refnum<k24>, error out=w412:errorcluster)  [unwired: 2 in, 1 out]
      n161 = property on="属性节点" class="CFXEnvelope"(reference=w413, error in=w412, "MessageBody"=w407) -> (reference out=w409:refnum<k24>, error out=w410:errorcluster, "MessageName"=w406:string)
      n162 = Close Reference(reference=w399, error in (no error)=w410) -> (error out=w398:errorcluster)
      n163 = property on="FaultOccurrenceId" class="Str"(error in=w398, "Value"="" ("ToString")) -> (error out=w397:errorcluster)  [unwired: 1 in, 1 out]
    }
    frame "OperatorActivated" {
      # "操作员"
      n164 = Unbundle By Name(w420) -> ("Operatorldentifer"=w419:string, "LoginName"=w418:string)
      n165 = constructor class="OperatorActivated"() -> (reference out=w433:refnum<k24>, error out=w424:errorcluster)  [unwired: 3 in, 1 out]
      n166 = constructor class="Operator"(error in=w424) -> (reference out=w432:refnum<k24>, error out=w429:errorcluster)  [unwired: 2 in, 1 out]
      n167 = property class="Operator"(reference=w432, error in=w429, "OperatorIdentifier"=w419, "LoginName"=w418) -> (reference out=w431:refnum<k24>, error out=w430:errorcluster)
      n168 = property on="属性节点" class="OperatorActivated"(reference=w433, error in=w430, "Operator"=w431) -> (reference out=w422:refnum<k24>, error out=w426:errorcluster)
      n169 = constructor class="CFXEnvelope"(error in=w426) -> (reference out=w428:refnum<k24>, error out=w427:errorcluster)  [unwired: 2 in, 1 out]
      n170 = property on="属性节点" class="CFXEnvelope"(reference=w428, error in=w427, "MessageBody"=w422) -> (reference out=w421:refnum<k24>, error out=w425:errorcluster, "MessageName"=w423:string)
    }
    frame "OperatorDeactivated" {
      # "操作员退出"
      n171 = Unbundle By Name(w436) -> ("Operatorldentifer"=w435:string, "LoginName"=w434:string)
      n172 = constructor class="OperatorDeactivated"() -> (reference out=w448:refnum<k24>, error out=w440:errorcluster)  [unwired: 3 in, 1 out]
      n173 = constructor class="Operator"(error in=w440) -> (reference out=w444:refnum<k24>, error out=w441:errorcluster)  [unwired: 2 in, 1 out]
      n174 = property class="Operator"(reference=w444, error in=w441, "OperatorIdentifier"=w435, "LoginName"=w434) -> (reference out=w443:refnum<k24>, error out=w442:errorcluster)
      n175 = property on="属性节点" class="OperatorDeactivated"(reference=w448, error in=w442, "Operator"=w443) -> (reference out=w445:refnum<k24>, error out=w439:errorcluster)
      n176 = constructor class="CFXEnvelope"() -> (reference out=w447:refnum<k24>, error out=w446:errorcluster)  [unwired: 3 in, 1 out]
      n177 = property on="属性节点" class="CFXEnvelope"(reference=w447, error in=w446, "MessageBody"=w445) -> (reference out=w438:refnum<k24>, "MessageName"=w437:string)  [unwired: 1 out]
    }
    frame "RecipeModified" {
      w462 = 4 items=["Unspecified", "NewRecipe", "NewRevision", "UpdatedGeometry", "UpdatedBOM", "PositionalCorrection", "RotationalCorrection", "VisionSystemCorrection", "RecipeDeleted"] ("Reason")
      # "设备首次生成一个新配方或已有配方发生修改时"
      n178 = Unbundle By Name(w453) -> ("Operatorldentifer"=w452:string, "LoginName"=w451:string, "RecipeName"=w450:string, "Revision"=w449:string)
      n179 = constructor class="RecipeModified"() -> (reference out=w467:refnum<k24>, error out=w455:errorcluster)  [unwired: 3 in, 1 out]
      n180 = constructor class="Operator"(error in=w455) -> (reference out=w464:refnum<k24>, error out=w463:errorcluster)  [unwired: 2 in, 1 out]
      n181 = property class="Operator"(reference=w464, error in=w463, "OperatorIdentifier"=w452, "LoginName"=w451) -> (reference out=w461:refnum<k24>, error out=w454:errorcluster)
      n182 = property on="属性节点" class="RecipeModified"(reference=w467, error in=w454, "RecipeName"=w450, "Revision"=w449, "ModifiedBy"=w461, "Reason"=w462) -> (reference out=w460:refnum<k24>, error out=w459:errorcluster)
      n183 = constructor class="CFXEnvelope"(error in=w459) -> (reference out=w466:refnum<k24>, error out=w465:errorcluster)  [unwired: 2 in, 1 out]
      n184 = property on="属性节点" class="CFXEnvelope"(reference=w466, error in=w465, "MessageBody"=w460) -> (reference out=w457:refnum<k24>, error out=w458:errorcluster, "MessageName"=w456:string)
    }
    frame "RecipeActived" {
      # "人工配方激活:当某个配方被激活时设备发送此事件型消息"
      n185 = Unbundle By Name(w470) -> ("RecipeName"=w469:string, "Revision"=w468:string)
      n186 = constructor class="RecipeActivated"(error in=w475) -> (reference out=w480:refnum<k24>, error out=w476:errorcluster)  [unwired: 2 in, 1 out]
      n187 = property on="属性节点" class="RecipeActivated"(reference=w480, error in=w476, "RecipeName"=w469, "Revision"=w468) -> (reference out=w477:refnum<k24>, error out=w474:errorcluster)
      n188 = constructor class="CFXEnvelope"(error in=w474) -> (reference out=w479:refnum<k24>, error out=w478:errorcluster)  [unwired: 2 in, 1 out]
      n189 = property on="属性节点" class="CFXEnvelope"(reference=w479, error in=w478, "MessageBody"=w477) -> (reference out=w473:refnum<k24>, error out=w471:errorcluster, "MessageName"=w472:string)
    }
    frame "ActivateRecipeRequest" {
      n190 = Unbundle By Name(w483) -> ("RecipeName"=w482:string, "Revision"=w481:string)
      n191 = constructor class="ActivateRecipeRequest"() -> (reference out=w490:refnum<k24>, error out=w488:errorcluster)  [unwired: 3 in, 1 out]
      n192 = property on="属性节点" class="ActivateRecipeRequest"(reference=w490, error in=w488, "RecipeName"=w482, "Revision"=w481) -> (reference out=w489:refnum<k24>, error out=w487:errorcluster)
      n193 = constructor class="CFXEnvelope"(error in=w487) -> (reference out=w492:refnum<k24>, error out=w491:errorcluster)  [unwired: 2 in, 1 out]
      n194 = property on="属性节点" class="CFXEnvelope"(reference=w492, error in=w491, "MessageBody"=w489) -> (reference out=w485:refnum<k24>, error out=w486:errorcluster, "MessageName"=w484:string)
    }
    frame "ActivateRecipeResponse" {
      w505 = 0 items=["Success", "PartialSuccess", "Failed", "Warning"] ("Result")
      n195 = constructor class="ActivateRecipeResponse"() -> (reference out=w509:refnum<k24>, error out=w496:errorcluster)  [unwired: 3 in, 1 out]
      n196 = case shown="True" TRUE {
        tunnel: ["Recipe not found" ("Message") "OK" ("Message")] -> w503
        frame False {
        }
        frame True {
        }
      }
      n197 = constructor class="RequestResult"(error in=w496) -> (reference out=w501:refnum<k24>, error out=w500:errorcluster)  [unwired: 2 in, 1 out]
      n198 = property class="RequestResult"(reference=w501, error in=w500, "Message"=w503, "Result"=w505, "ResultCode"=0) -> (reference out=w506:refnum<k24>, error out=w499:errorcluster)
      n199 = property on="属性节点" class="ActivateRecipeResponse"(reference=w509, error in=w499, "Result"=w506) -> (reference out=w507:refnum<k24>, error out=w495:errorcluster)
      n200 = constructor class="CFXEnvelope"(error in=w495) -> (reference out=w493:refnum<k24>, error out=w508:errorcluster)  [unwired: 2 in, 1 out]
      n201 = property on="属性节点" class="CFXEnvelope"(reference=w493, error in=w508, "MessageBody"=w507) -> (reference out=w498:refnum<k24>, error out=w494:errorcluster, "MessageName"=w497:string)
    }
  }
  "MessageName" <- w8
  n202 = invoke class="CFXEnvelope" method="ToJson"(reference=w6, error in=w4, "formatted"=TRUE) -> (reference out=→"new reference":refnum<k24>, error out=→"Error Out":errorcluster, "ToJson"=→"Message":string)  [unwired: 1 in, 1 out]
